vi "FRC_extract text between.vi"(0 "string":string, 5 "after this text":string, 7 "before this text":string) -> (4 "leftover text":string, 6 "after text":string, 8 "extracted text":string, 10 "before text":string)   [LabVIEW 2023, in "GettingStartedWindow.lvlib"]
uses:
  <resource>/modes/FRC/GSW/GettingStartedWindow.lvlib
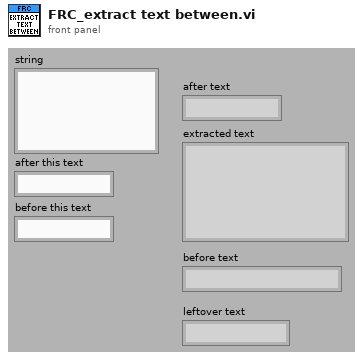
[diagram p1: front panel]
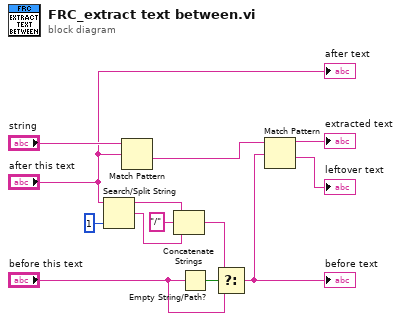
[diagram p0: block diagram]
diagram:
  n1 = Search/Split String(string="after this text", offset (0)=1) -> (substring before match=w7:string, match + rest of string=w5:string)  [unwired: 1 in, 1 out]
  n2 = Match Pattern(string="string", regular expression="after this text") -> (after substring=w12:string)  [unwired: 1 in, 3 out]
  n3 = Concatenate Strings(w7, "/" ("Substring"), w5) -> (w4:string)
  n4 = Empty String/Path?(string/path="before this text") -> (empty?=w9:bool)
  n5 = Select(t=w4, s=w9, f="before this text") -> (s? t:f=w2:string)
  "before text" <- w2
  n6 = Match Pattern(string=w12, regular expression=w2) -> (before substring=→"extracted text":string, after substring=→"leftover text":string)  [unwired: 1 in, 2 out]
  "after text" <- "after this text"
